vi "PictureControl_MouseUp.vi"(7 "Finalize Movement":bool, 8 "error in":errorcluster, 10 "Coords":T5, 11 "Data in":T1={"Class"={"Ants"=refnum, "Layer"=refnum, "Templates"=refnum, "Icon"=refnum, "Glyph"=refnum, "Settings"=refnum, "Tools"=refnum, "History"=refnum}, "Ref"={"Add Layer"=refnum, "Remove Layer"=refnum, "Line Text"=[], "Body Text Spec"=refnum, "DNL_Font"=refnum, "glyph path str"=refnum, "templates path str"=refnum, "Arrow Up"=refnum, "Arrow Down"=refnum, "IE VI Ref"=refnum, "Glyphs tree"=refnum, "Templates tree"=refnum, "Layer Icon Text"=refnum, "Layer Template"=refnum, "Body Text"=refnum, "Search Templates"=refnum, "TextMarker"=refnum, "Tab Control"=refnum, "Search Glyphs"=refnum, "Line Color"=refnum, "DNL_Glyphs []"=refnum, "Fill Color"=refnum, "Tools"=refnum, "Icon"=refnum, "Preview"=refnum, "Ants"=refnum, "Terminals"=refnum, "menu reference"=refnum, "LayerNames"=[], "GlyphLoadAnimation"=refnum, "TemplateLoadAnimation"=refnum, "refreshGlyphs"=refnum, "refreshTemplates"=refnum}, "Support"={"AntsRect"={"left"=0, "top"=0, "right"=0, "bottom"=0}, "Mouse Move Coords"={"Horizontal"=0, "Vertical"=0}, "Mouse Down Coords"={"Horizontal"=0, "Vertical"=0}, "Temp Coord"={"Horizontal"=0, "Vertical"=0}, "Action"=enum."Default", "Edge Color"=4914962, "Fill Color"=16860, "Mouse Down?"=FALSE, "Draft Mode?"=FALSE, "Temp Icon"=bytes[3102], "CTRL Pressed"=FALSE, "Move Selection?"=FALSE, "AntsRect Orig"={"left"=0, "top"=0, "right"=0, "bottom"=0}, "Text"="", "TM Set?"=FALSE, "Mouse inside icon?"=FALSE, "Tool (old value)"=0, "Pencil Move Color"=0, "Swap Colors?"=FALSE, "Shift pressed?"=FALSE}}) -> (0 "error out":errorcluster, 3 "Data out":T1={"Class"={"Ants"=refnum, "Layer"=refnum, "Templates"=refnum, "Icon"=refnum, "Glyph"=refnum, "Settings"=refnum, "Tools"=refnum, "History"=refnum}, "Ref"={"Add Layer"=refnum, "Remove Layer"=refnum, "Line Text"=[], "Body Text Spec"=refnum, "DNL_Font"=refnum, "glyph path str"=refnum, "templates path str"=refnum, "Arrow Up"=refnum, "Arrow Down"=refnum, "IE VI Ref"=refnum, "Glyphs tree"=refnum, "Templates tree"=refnum, "Layer Icon Text"=refnum, "Layer Template"=refnum, "Body Text"=refnum, "Search Templates"=refnum, "TextMarker"=refnum, "Tab Control"=refnum, "Search Glyphs"=refnum, "Line Color"=refnum, "DNL_Glyphs []"=refnum, "Fill Color"=refnum, "Tools"=refnum, "Icon"=refnum, "Preview"=refnum, "Ants"=refnum, "Terminals"=refnum, "menu reference"=refnum, "LayerNames"=[], "GlyphLoadAnimation"=refnum, "TemplateLoadAnimation"=refnum, "refreshGlyphs"=refnum, "refreshTemplates"=refnum}, "Support"={"AntsRect"={"left"=0, "top"=0, "right"=0, "bottom"=0}, "Mouse Move Coords"={"Horizontal"=0, "Vertical"=0}, "Mouse Down Coords"={"Horizontal"=0, "Vertical"=0}, "Temp Coord"={"Horizontal"=0, "Vertical"=0}, "Action"=enum."Default", "Edge Color"=4914962, "Fill Color"=16860, "Mouse Down?"=FALSE, "Draft Mode?"=FALSE, "Temp Icon"=bytes[3102], "CTRL Pressed"=FALSE, "Move Selection?"=FALSE, "AntsRect Orig"={"left"=0, "top"=0, "right"=0, "bottom"=0}, "Text"="", "TM Set?"=FALSE, "Mouse inside icon?"=FALSE, "Tool (old value)"=0, "Pencil Move Color"=0, "Swap Colors?"=FALSE, "Shift pressed?"=FALSE}})   [LabVIEW 2020]
uses:
  Class/Ants/Ants.lvclass
  Class/FakedArray/FakedArray.lvclass
  vi.lib/LabVIEW Icon API/lv_icon/Classes/Icon/Icon.lvclass
  Class/Icon Library/Glyph.lvclass
  Class/Settings/Settings.lvclass
  Class/Tools/Tools Paint.lvclass
  History/History/History.lvclass
  Controls/SupportClass_Action.ctl
  History/History.lvlib
  <vilib>/Utility/miscctls.llb/LVPoint32TypeDef.ctl
  vi.lib/LabVIEW Icon API/lv_icon/Controls/IEColor.ctl
  Controls/Support Cluster.ctl
  lv_icon.lvlib
  Controls/References Cluster.ctl
  Controls/IE Classes.ctl
  Controls/Global Data.ctl
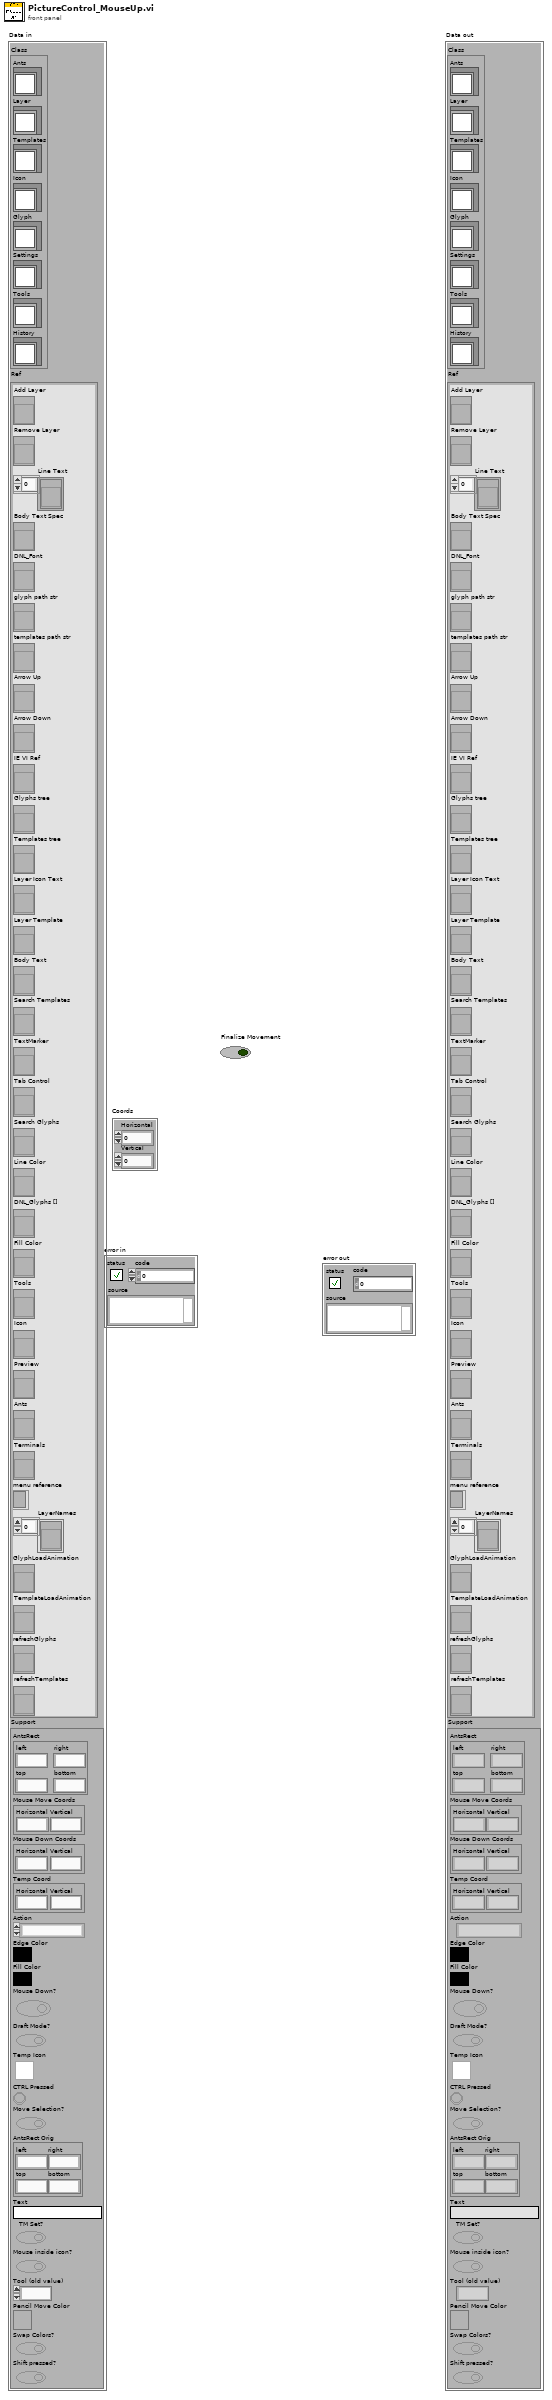
[diagram p1: front panel]
types:
  T1 = typedef "lv_icon.lvlib/Global Data.ctl" = cluster{"Class":T2, "Ref":T3, "Support":T4}
  T2 = typedef "lv_icon.lvlib/IE Classes.ctl" = cluster{"Ants":refnum<class "Ants.lvclass">, "Layer":refnum<class "FakedArray.lvclass">, "Templates":refnum<class "FakedArray.lvclass">, "Icon":refnum<class "Icon.lvclass">, "Glyph":refnum<class "Glyph.lvclass">, "Settings":refnum<class "Settings.lvclass">, "Tools":refnum<class "Tools Paint.lvclass">, "History":refnum<class "History.lvclass">}
  T3 = typedef "lv_icon.lvlib/References Cluster.ctl" = cluster{"Add Layer":refnum<vi>, "Remove Layer":refnum<vi>, "Line Text":refnum<vi>[], "Body Text Spec":refnum<vi>, "DNL_Font":refnum<vi>, "glyph path str":refnum<vi>, "templates path str":refnum<vi>, "Arrow Up":refnum<vi>, "Arrow Down":refnum<vi>, "IE VI Ref":refnum<vi>, "Glyphs tree":refnum<vi>, "Templates tree":refnum<vi>, "Layer Icon Text":refnum<vi>, "Layer Template":refnum<vi>, "Body Text":refnum<vi>, "Search Templates":refnum<vi>, "TextMarker":refnum<vi>, "Tab Control":refnum<vi>, "Search Glyphs":refnum<vi>, "Line Color":refnum<vi>, "DNL_Glyphs []":refnum<vi>, "Fill Color":refnum<vi>, "Tools":refnum<vi>, "Icon":refnum<vi>, "Preview":refnum<vi>, "Ants":refnum<vi>, "Terminals":refnum<vi>, "menu reference":refnum<k9>, "LayerNames":refnum<vi>[], "GlyphLoadAnimation":refnum<vi>, "TemplateLoadAnimation":refnum<vi>, "refreshGlyphs":refnum<vi>, "refreshTemplates":refnum<vi>}
  T4 = typedef "lv_icon.lvlib/Support Cluster.ctl" = cluster{"AntsRect":cluster{"left":i16, "top":i16, "right":i16, "bottom":i16}, "Mouse Move Coords":T5, "Mouse Down Coords":T5, "Temp Coord":T5, "Action":T6, "Edge Color":T7, "Fill Color":T7, "Mouse Down?":bool, "Draft Mode?":bool, "Temp Icon":picture, "CTRL Pressed":bool, "Move Selection?":bool, "AntsRect Orig":cluster{"left":i16, "top":i16, "right":i16, "bottom":i16}, "Text":string, "TM Set?":bool, "Mouse inside icon?":bool, "Tool (old value)":u32, "Pencil Move Color":u32, "Swap Colors?":bool, "Shift pressed?":bool}
  T5 = typedef "LVPoint32TypeDef.ctl" = cluster{"Horizontal":i32, "Vertical":i32}
  T6 = typedef "SupportClass_Action.ctl" = enum16{"Default", "Move Selection", "Glyph Library", "Tool"}
  T7 = typedef "IEColor.ctl" = u32
  T8 = cluster{"left":i16, "top":i16, "right":i16, "bottom":i16}
  T9 = cluster{"Horizontal":i32, "Vertical":i32, "Vertical 2":i32, "Vertical 3":i32}
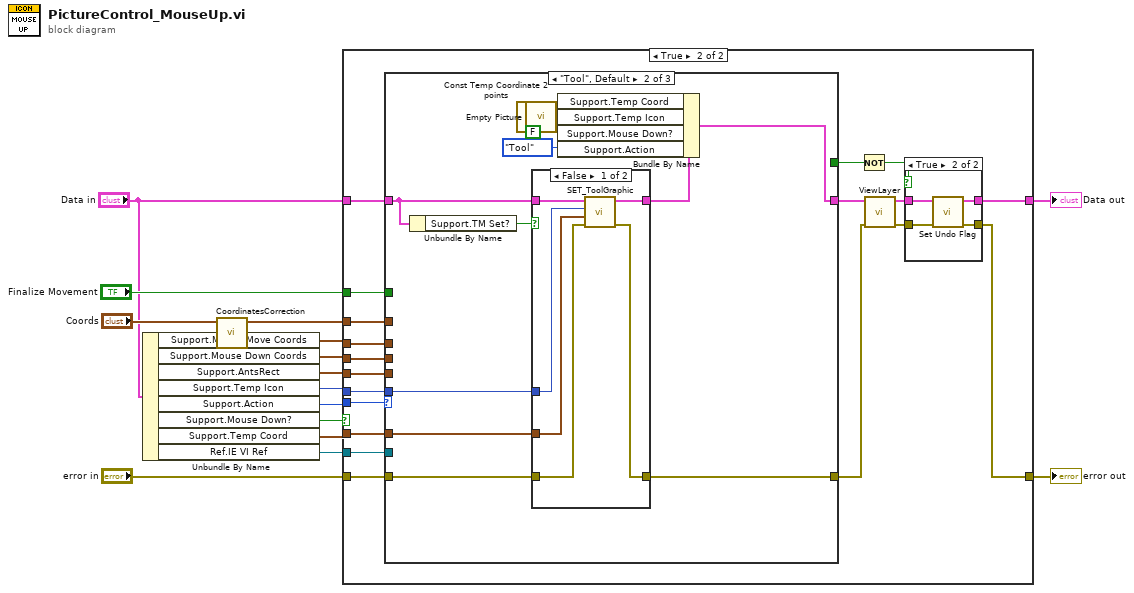
[diagram p0: block diagram]
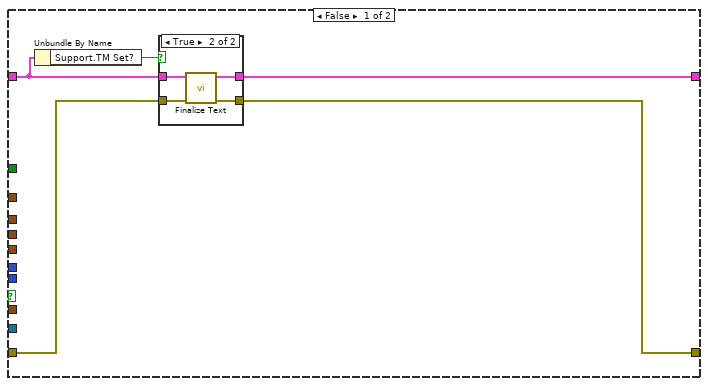
[diagram p2: hidden frame]
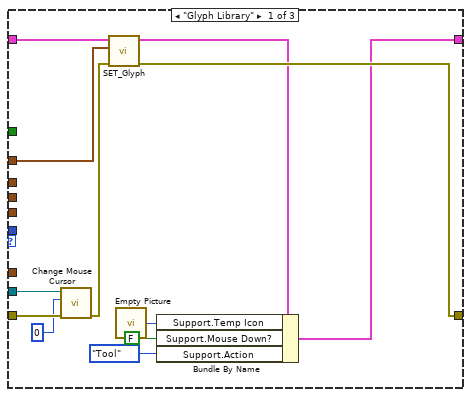
[diagram p5: hidden frame]
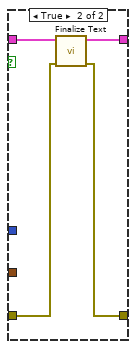
[diagram p6: hidden frame]
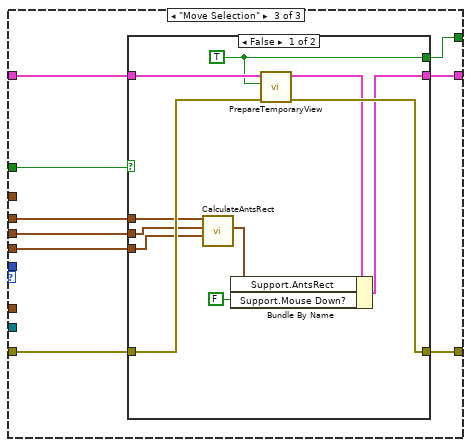
[diagram p7: hidden frame]
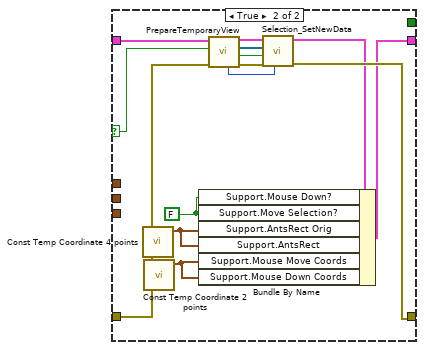
[diagram p8: hidden frame]
diagram:
  n1 = Unbundle By Name("Data in") -> ("Support.Mouse Move Coords"=w4:T5, "Support.Mouse Down Coords"=w5:T5, "Support.AntsRect"=w6:T8, "Support.Temp Icon"=w11:picture, "Support.Action"=w9:T6, "Support.Mouse Down?"=w10:bool, "Support.Temp Coord"=w13:T5, "Ref.IE VI Ref"=w3:refnum<vi>)
  n2 = call "CoordinatesCorrection.vi"("Coordinates In"="Coords") -> ("Corrected Out"=w12:T5)  [unwired: 10 out]
  n3 = case shown="True" w10 {
    tunnel: w9 -> [_ w41]
    tunnel: "error in" -> [w20 w45]
    tunnel: w11 -> [_ w40]
    tunnel: w12 -> [_ w39]
    tunnel: [w19 w42] -> w14
    tunnel: w13 -> [_ w38]
    tunnel: "Finalize Movement" -> [_ w37]
    tunnel: w6 -> [_ w36]
    tunnel: w5 -> [_ w35]
    tunnel: w4 -> [_ w34]
    tunnel: "Data in" -> [w17 w33]
    tunnel: [w16 w29] -> w1
    tunnel: w3 -> [_ w31]
    frame False {
      n4 = Unbundle By Name(w17) -> ("Support.TM Set?"=w18:bool)
      n5 = case shown="True" w18 {
        tunnel: w17 -> [w21 w24]
        tunnel: [w21 w23] -> w16
        tunnel: w20 -> [w22 w26]
        tunnel: [w22 w25] -> w19
        frame False {
        }
        frame True {
          n6 = call "Finalize Text.vi"("error in (no error)"=w26, "Data in"=w24) -> ("error out"=w25:errorcluster, "Data out"=w23:T1)  [unwired: 8 in]
        }
      }
    }
    frame True {
      n7 = case shown="\"Tool\", Default" w41 {
        tunnel: w45 -> [w62 w74 w94]
        tunnel: w40 -> [_ w73 _]
        tunnel: w39 -> [w60 _ _]
        tunnel: [w52 w67 w92] -> w32
        tunnel: [w63 w75 w93] -> w44
        tunnel: w38 -> [_ w72 _]
        tunnel: w37 -> [_ _ w91]
        tunnel: w36 -> [_ _ w88]
        tunnel: w35 -> [_ _ w89]
        tunnel: w34 -> [_ _ w90]
        tunnel: w33 -> [w56 w65 w87]
        tunnel: w31 -> [w54 _ _]
        tunnel: [_ _ w86] -> w28
        frame "Glyph Library" {
          n8 = call "Change Mouse Cursor.vi"("error in (no error)"=w62, "icon"=u16 0, "VI reference (current VI)"=w54) -> ("error out"=w61:errorcluster)  [unwired: 8 out]
          n9 = call "SET_Glyph.vi"("error in"=w61, "Coordinates"=w60, "Data in"=w56) -> ("error out"=w63:errorcluster, "Data out"=w53:T1)  [unwired: 7 out]
          n10 = call "Empty Picture"() -> ("empty picture"=w57:picture)
          n11 = Bundle By Name(cluster=w53, "Support.Temp Icon"=w57, "Support.Mouse Down?"=FALSE ("Mouse Down?"), "Support.Action"=SupportClass_Action."Tool" ("Action")) -> (w52:T1)
        }
        frame "Tool", Default {
          n12 = Unbundle By Name(w65) -> ("Support.TM Set?"=w64:bool)
          n13 = call "Const Temp Coordinate 2 points.vi"() -> ("Const Temp Coordinate"=w71:T5)  [unwired: 11 out]
          n14 = call "Empty Picture"() -> ("empty picture"=w70:picture)
          n15 = case shown="False" w64 {
            tunnel: [w81 w82] -> w75
            tunnel: w74 -> [w80 w83]
            tunnel: w73 -> [w79 _]
            tunnel: w72 -> [w78 _]
            tunnel: [w77 w84] -> w66
            tunnel: w65 -> [w76 w85]
            frame False {
              n16 = call "SET_ToolGraphic.vi"("error in"=w80, "Temp Coord"=w78, "Temp Icon"=w79, "Data in"=w76) -> ("error out"=w81:errorcluster, "Data out"=w77:T1)  [unwired: 6 out]
            }
            frame True {
              n17 = call "Finalize Text.vi"("error in (no error)"=w83, "Data in"=w85) -> ("error out"=w82:errorcluster, "Data out"=w84:T1)  [unwired: 8 in]
            }
          }
          n18 = Bundle By Name(cluster=w66, "Support.Temp Coord"=w71, "Support.Temp Icon"=w70, "Support.Mouse Down?"=FALSE ("Mouse Down?"), "Support.Action"=SupportClass_Action."Tool" ("Action")) -> (w67:T1)
        }
        frame "Move Selection" {
          n19 = case shown="False" w91 {
            selector: w91 -> [_ w113]
            tunnel: w94 -> [w105 w118]
            tunnel: [w104 w117] -> w93
            tunnel: [w96 w112] -> w92
            tunnel: w90 -> [w102 _]
            tunnel: w89 -> [w101 _]
            tunnel: w88 -> [w100 _]
            tunnel: w87 -> [w98 w108]
            tunnel: [w95 _] -> w86
            frame False {
              w95 = TRUE ("Valid Selection?")
              n20 = call "CalculateAntsRect.vi"("AntsRect"=w100, "Mouse Down Coords"=w101, "Mouse Move Coords"=w102) -> ("Rect"=w99:cluster{i32, i32, i32, i32})  [unwired: 8 out]
              n21 = call "PrepareTemporaryView.vi"("error in (no error)"=w105, "Valid Selection?"=w95, "Data in"=w98) -> ("error out"=w104:errorcluster, "Data out"=w97:T1)  [unwired: 2 in, 5 out]
              n22 = Bundle By Name(cluster=w97, "Support.AntsRect"=w99, "Support.Mouse Down?"=FALSE ("Mouse Down?")) -> (w96:T1)
            }
            frame True {
              w111 = FALSE ("Move Selection?")
              n23 = call "Const Temp Coordinate 4 points.vi"() -> ("Const Temp Coordinate"=w110:T9)  [unwired: 11 out]
              n24 = call "Const Temp Coordinate 2 points.vi"() -> ("Const Temp Coordinate"=w109:T5)  [unwired: 11 out]
              n25 = call "PrepareTemporaryView.vi"("error in (no error)"=w118, "Valid Selection?"=w113, "Data in"=w108) -> ("error out"=w119:errorcluster, "Highlighted?"=w115:bool, "All Layers out"=w116:refnum<class "Layer.lvclass">[], "Data out"=w107:T1, "#Active Layer"=w114:i32)  [unwired: 2 in, 2 out]
              n26 = call "Selection_SetNewData.vi"("#Active Layer"=w114, "error in"=w119, "Highlighted?"=w115, "All Layers In"=w116, "Data in"=w107) -> ("error out"=w117:errorcluster, "Data out"=w106:T1)  [unwired: 1 in, 3 out]
              n27 = Bundle By Name(cluster=w106, "Support.Mouse Down?"=w111, "Support.Move Selection?"=w111, "Support.AntsRect Orig"=w110, "Support.AntsRect"=w110, "Support.Mouse Move Coords"=w109, "Support.Mouse Down Coords"=w109) -> (w112:T1)
            }
          }
        }
      }
      n28 = Not(x=w28) -> (.not. x?=w27:bool)
      n29 = call "ViewLayer.vi"("error in (no error)"=w44, "Data in"=w32) -> ("error out"=w43:errorcluster, "Data out"=w30:T1)  [unwired: 3 in, 5 out]
      n30 = case shown="True" w27 {
        tunnel: w43 -> [w47 w51]
        tunnel: [w47 w50] -> w42
        tunnel: w30 -> [w46 w49]
        tunnel: [w46 w48] -> w29
        frame False {
        }
        frame True {
          n31 = call "Set Undo Flag.vi"("error in"=w51, "Data in"=w49) -> ("error out"=w50:errorcluster, "Data out"=w48:T1)  [unwired: 8 in]
        }
      }
    }
  }
  "error out" <- w14
  "Data out" <- w1
